vi "Update terminal.vi"(11 "VI in":refnum<vi>) -> (0 "error out":errorcluster, 2 "change?":bool)   [LabVIEW 2019]
uses:
  <vilib>/Utility/traverseref.llb/TRef TravTarget.ctl
  <vilib>/numeric/LVNumericRepresentation.ctl
  <vilib>/Utility/traverseref.llb/VI Scripting - Traverse.lvlib
panel:
  in  "error in (no error)":errorcluster
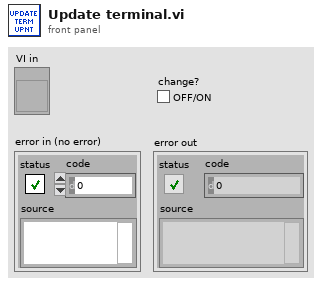
[diagram p1: front panel]
types:
  T1 = typedef "TRef TravTarget.ctl" = enum16{"FP", "BD", "Other"}
  T2 = typedef "LVNumericRepresentation.ctl" = enum32{"Extended Precision", "Double Precision", "Single Precision", "Long", "Word", "Byte", "Unsigned Long", "Unsigned Word", "Unsigned Byte", "Complex Extended", "Complex Double", "Complex Single", "Quad", "Unsigned Quad", "Fixed-Point"}
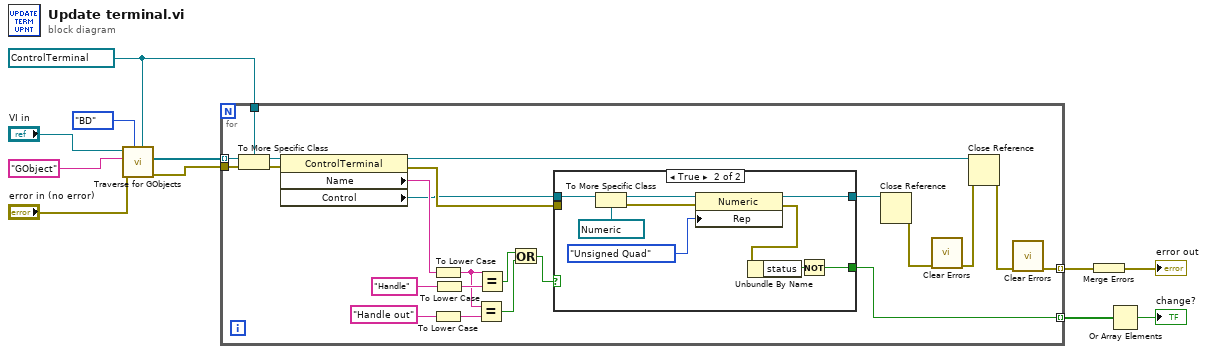
[diagram p0: block diagram]
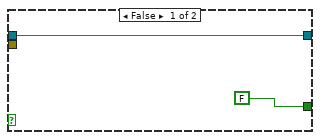
[diagram p2: hidden frame]
diagram:
  w8 = refnum<vi> refnum ("Other Refnum")
  n1 = call <vilib>:"Traverse for GObjects.vi"("Other Refnum"=w8, "Traverse Target"=TRef_TravTarget."BD", "error in (no error)"="error in (no error)", "Class Name"="GObject", "VI Refnum"="VI in") -> ("error out"=w7:errorcluster, "References"=w10:refnum<vi>[])  [unwired: 3 in, 2 out]
  n2 = for {
    tunnel: w10 -> [w32] mode=indexing
    tunnel: w8 -> [w34]
    tunnel: w7 -> [w27]
    tunnel: [w18] -> w5 mode=indexing
    tunnel: [w22] -> w3 mode=indexing
    n3 = To More Specific Class(target class=w34, reference=w32, error in=w27) -> (specific class reference=w33:refnum<vi>, error out=w28:errorcluster)
    n4 = property class="ControlTerminal"(reference=w33, error in=w28) -> (reference out=w19:refnum<vi>, error out=w25:errorcluster, "Name"=w31:string, "Control"=w24:refnum<vi>)
    n5 = To Lower Case(string=w31) -> (all lower case string=w15:string)
    n6 = To Lower Case(string="Handle out" ("y")) -> (all lower case string=w17:string)
    n7 = To Lower Case(string="Handle" ("y")) -> (all lower case string=w29:string)
    n8 = Equal?(x=w15, y=w17) -> (x = y?=w14:bool)
    n9 = Equal?(x=w15, y=w29) -> (x = y?=w13:bool)
    n10 = Or(x=w13, y=w14) -> (x .or. y?=w12:bool)
    n11 = case shown="True" w12 {
      tunnel: w24 -> [w36 w44]
      tunnel: [w36 w41] -> w26
      tunnel: [FALSE w37] -> w18
      tunnel: w25 -> [_ _]
      frame False {
      }
      frame True {
        n12 = To More Specific Class(target class=refnum<vi> refnum ("Other Refnum"), reference=w44) -> (specific class reference=w43:refnum<vi>, error out=w40:errorcluster)  [unwired: 1 in]
        n13 = property class="Numeric"(reference=w43, error in=w40, "Rep"=LVNumericRepresentation."Unsigned Quad" ("Representation")) -> (reference out=w41:refnum<vi>, error out=w38:errorcluster)
        n14 = Unbundle By Name(w38) -> ("status"=w39:bool)
        n15 = Not(x=w39) -> (.not. x?=w37:bool)
      }
    }
    n16 = Close Reference(reference=w26) -> (error out=w21:errorcluster)  [unwired: 1 in]
    n17 = call <vilib>:"Clear Errors.vi"("error in (no error)"=w21) -> ("error out"=w20:errorcluster)  [unwired: 5 in, 1 out]
    n18 = Close Reference(reference=w19, error in (no error)=w20) -> (error out=w23:errorcluster)
    n19 = call <vilib>:"Clear Errors.vi"("error in (no error)"=w23) -> ("error out"=w22:errorcluster)  [unwired: 5 in, 1 out]
  }
  n20 = Merge Errors(w3) -> (→"error out":errorcluster)
  n21 = Or Array Elements(Boolean array=w5) -> (logical OR=→"change?":bool)
